vi "MQTT Data Stream - Write Packet.vi"(0 "TCP Network Connection in":refnum<k5>, 1 "QoS":T2, 2 "Retain":bool, 5 "MessageType":T1, 7 "packet data":u8[](array[numeric]), 9 "TCP Timeout":i32=25000, 11 "error in (no error)":errorcluster, 12 "DUP":bool) -> (4 "TCP Network Connection out":refnum<k5>, 6 "DEBUG":string, 15 "error out":errorcluster)   [LabVIEW 2019, in "KoRE-MQTT.lvlib"]
doc: "Copyright (c) 2026 KoRElibs.com\nSPDX-License-Identifier: EUPL-1.2\n\nThis VI is licensed under the European Union Public License (EUPL) Version 1.2. You may use this VI unmodified in proprietary works. If you distribute a modified version of this file, the modified file must be released under the EUPL-1.2. Full license: https://joinup.ec.europa.eu/asset/eupl/eupl/1.2/\n\nCopyright (c) 2025 KoRElibs.com\nSPDX-License-Identifier: EUPL-1.2\n\nThis VI is licensed under the European Union Public License (EUPL) Version 1.2. You may use this VI unmodified in proprietary works. If you distribute a modified version of this file, the modified file must be released under the EUPL-1.2. Full license: https://joinup.ec.europa.eu/asset/eupl/eupl/1.2/"
uses:
  KoRE-MQTT.lvlib
  Public/TypeDefs/MQTT QoS Level.ctl
  TypeDefs/MQTT Packet - Type.ctl
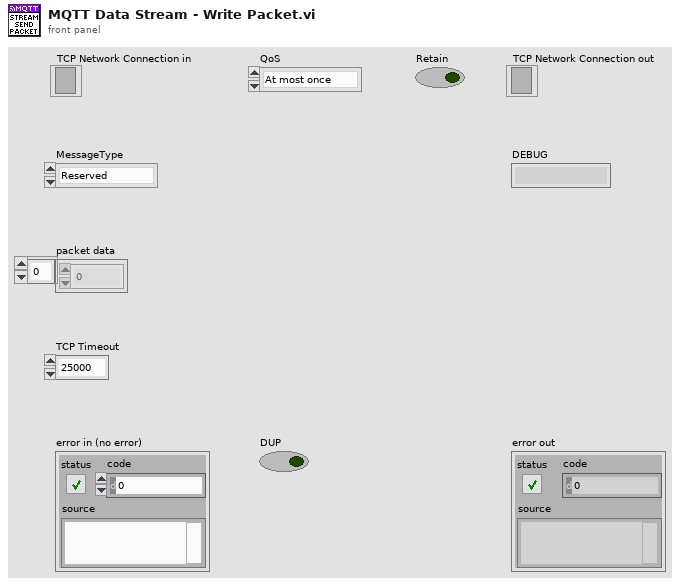
[diagram p1: front panel]
types:
  T1 = typedef "KoRE-MQTT.lvlib/MQTT Packet - Type.ctl" = enum32{"Reserved", "CONNECT", "CONNACK", "PUBLISH", "PUBACK", "PUBREC", "PUBREL", "PUBCOMP", "SUBSCRIBE", "SUBACK", "UNSUBSCRIBE", "UNSUBACK", "PINGREQ", "PINGRESP", "DISCONNECT", "AUTH"}
  T2 = typedef "KoRE-MQTT.lvlib/MQTT QoS Level.ctl" = enum8{"At most once", "At least once", "Exactly once"}
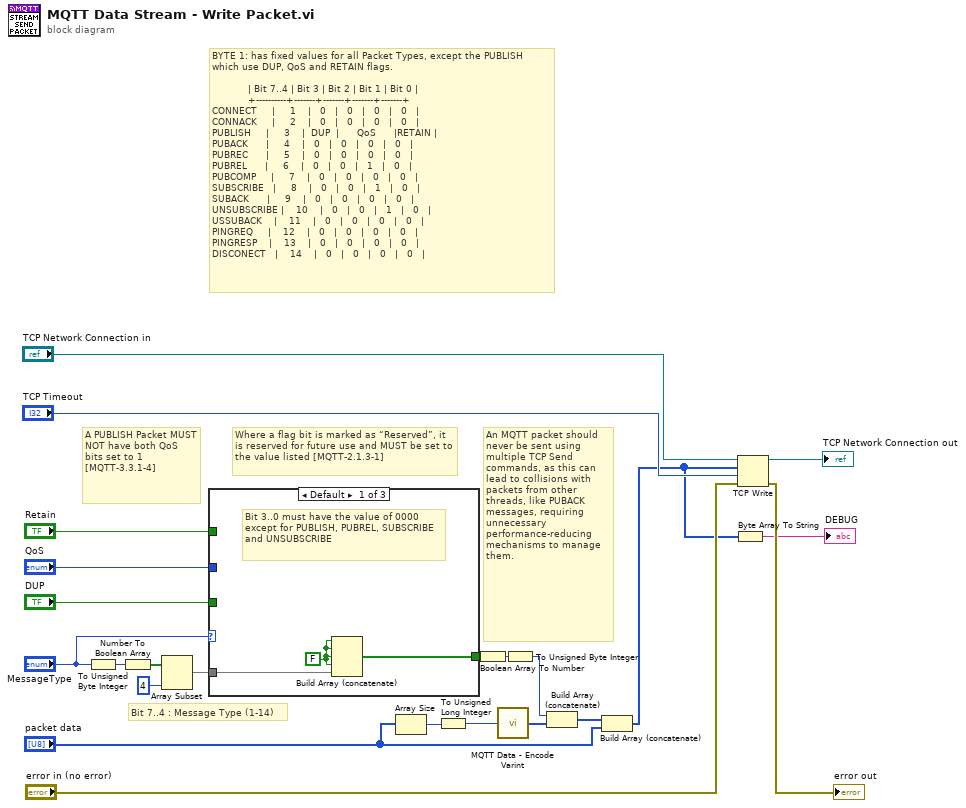
[diagram p0: block diagram]
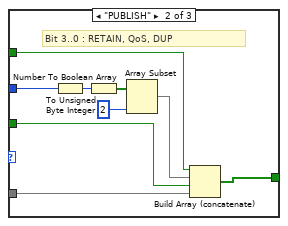
[diagram p2: hidden frame]
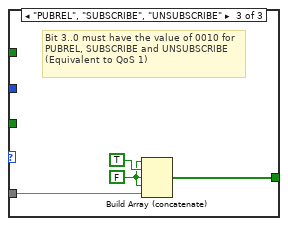
[diagram p3: hidden frame]
diagram:
  # "BYTE 1: has fixed values for all Packet Types, except the PUBLISH which use DUP, QoS and RETAIN flags.\n\n            | Bit 7..4 | Bit 3 | Bit 2 | Bit 1 | Bit 0 |\n            +----------+-------+-------+-------+-------+\nCONNECT     |     1    |   0   |   0   |   0   |   0   |\nCONNACK     |     2    |   0   |   0   |   0   |   0   |\nPUBLISH     |     3    |  DUP  |      QoS      |RETAIN |\nPUBACK      |     4    |   0   |   0   |   0   |   0   |\nPUBREC      |     5    |   0   |   0   |   0   |   0   |\nPUBREL      |     6    |   0   |   0   |   1   |   0   |\nPUBCOMP     |     7    |   0   |   0   |   0   |   0   |\nSUBSCRIBE   |     8    |   0   |   0   |   1   |   0   |\nSUBACK      |     9    |   0   |   0   |   0   |   0   |\nUNSUBSCRIBE |    10    |   0   |   0   |   1   |   0   |\nUSSUBACK    |    11    |   0   |   0   |   0   |   0   |\nPINGREQ     |    12    |   0   |   0   |   0   |   0   |\nPINGRESP    |    13    |   0   |   0   |   0   |   0   |\nDISCONECT   |    14    |   0   |   0   |   0   |   0   |"
  # "A PUBLISH Packet MUST NOT have both QoS bits set to 1 [MQTT-3.3.1-4]"
  # "Bit 7..4 : Message Type (1-14)"
  # "An MQTT packet should never be sent using multiple TCP Send commands, as this can lead to collisions with packets from other threads, like PUBACK messages, requiring unnecessary performance-reducing mechanisms to manage them."
  # "Where a flag bit is marked as “Reserved”, it is reserved for future use and MUST be set to the value listed [MQTT-2.1.3-1]"
  n1 = To Unsigned Byte Integer(number="MessageType") -> (unsigned 8bit integer=w12:u8)
  n2 = Number To Boolean Array(number=w12) -> (Boolean array=w11:bool[])
  n3 = Array Subset(array=w11, length=4) -> (w7:bool[])  [unwired: 1 in]
  n4 = case shown="Default" "MessageType" {
    tunnel: [w24 w35 w36] -> w6
    tunnel: "QoS" -> [_ w30 _]
    tunnel: w7 -> [w25 w34 w39]
    tunnel: "DUP" -> [_ w28 _]
    tunnel: "Retain" -> [_ w27 _]
    frame Default {
      w26 = FALSE
      # "Bit 3..0 must have the value of 0000 except for PUBLISH, PUBREL, SUBSCRIBE and UNSUBSCRIBE"
      n5 = Build Array (concatenate)(w26, w26, w26, w26, w25) -> (w24:bool[])
    }
    frame "PUBLISH" {
      # "Bit 3..0 : RETAIN, QoS, DUP"
      n6 = To Unsigned Byte Integer(number=w30) -> (unsigned 8bit integer=w31:u8)
      n7 = Number To Boolean Array(number=w31) -> (Boolean array=w32:bool[])
      n8 = Array Subset(array=w32, length=2) -> (w29:bool[])  [unwired: 1 in]
      n9 = Build Array (concatenate)(w27, w29, w28, w34) -> (w35:bool[])
    }
    frame "PUBREL", "SUBSCRIBE", "UNSUBSCRIBE" {
      w37 = FALSE
      # "Bit 3..0 must have the value of 0010 for PUBREL, SUBSCRIBE and UNSUBSCRIBE (Equivalent to QoS 1)"
      n10 = Build Array (concatenate)(w37, TRUE, w37, w37, w39) -> (w36:bool[])
    }
  }
  n11 = Array Size(array="packet data") -> (size(s)=w3:i32)
  n12 = To Unsigned Long Integer(number=w3) -> (unsigned 32bit integer=w4:u32)
  n13 = Boolean Array To Number(Boolean array=w6) -> (number=w9:u32)
  n14 = call "MQTT Data - Encode Varint.vi"("Value"=w4) -> ("encoded value"=w5:u8[])  [unwired: 14 in]
  n15 = To Unsigned Byte Integer(number=w9) -> (unsigned 8bit integer=w8:u8)
  n16 = Build Array (concatenate)(w8, w5) -> (w2:u8[])
  n17 = Build Array (concatenate)(w2, "packet data") -> (w17:u8[])
  n18 = Byte Array To String(unsigned byte array=w17) -> (string=→"DEBUG":string)
  n19 = TCP Write(connection ID="TCP Network Connection in", data in=w17, error in (no error)="error in (no error)", 9:"TCP Timeout") -> (connection ID out=→"TCP Network Connection out":refnum<k5>, error out=→"error out":errorcluster)  [unwired: 1 out]
